vi "Import Export - Import from XML File.vi"(8 "error in":errorcluster, 10 "Configuration File Path":path, 11 "Item Ref in":T1 format="%.0x") -> (0 "error out":errorcluster, 3 "Item Ref out":T1 format="%.0x", 4 "xml string":string)   [LabVIEW 2017, in "PXImc System Explorer.lvlib"]
uses:
  PXImc System Explorer.lvlib
  <vilib>/NI Veristand/Custom Device API/Custom Device Item Ref.ctl
  <vilib>/NI/NI VeriStand Custom Device Import and Export Tool/ImportExport.lvlib
  <vilib>/NI VeriStand/Custom Device API/Custom Device API.lvlib
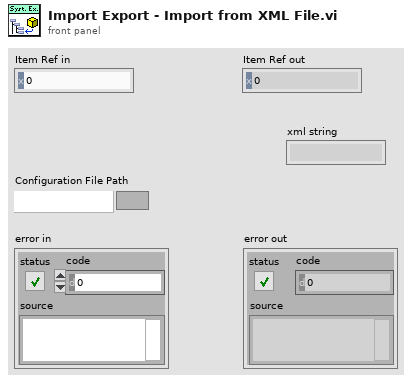
[diagram p1: front panel]
types:
  T1 = typedef "Custom Device API.lvlib/Custom Device Item Ref.ctl" = u64
  T2 = typedef "Advanced System Definition.lvlib/SysDef.Export.ctl" = cluster{"Version":string, "Tree":T3[]}
  T3 = typedef "Advanced System Definition.lvlib/TreeItem.ctl" = cluster{"Item Info":T4, "Parent Path":string[], "Properties":T9[]}
  T4 = typedef "Advanced System Definition.lvlib/TreeItem.Info.ctl" = cluster{"Name":string, "Description":string, "GUID":string, "Is Channel":bool, "Channel":T5, "Is Waveform":bool, "Waveform":T7}
  T5 = typedef "Custom Device API.lvlib/Custom Device Channel.ctl" = cluster{"Type":T6, "Units":string, "Default Value":dbl, "Faultable":bool, "Scalable":bool}
  T6 = typedef "Custom Device API.lvlib/Custom Device Channel Type.ctl" = enum16{"Input", "Output"}
  T7 = typedef "Custom Device API.lvlib/Custom Device Waveform.ctl" = cluster{"Data Type":T8, "Units":string}
  T8 = typedef "Custom Device API.lvlib/Custom Device Waveform DataType.ctl" = enum16{"Double", "Complex Double"}
  T9 = typedef "Advanced System Definition.lvlib/TreeItem.Property.ctl" = cluster{"Name":string, "Type":i32, "Value":variant}
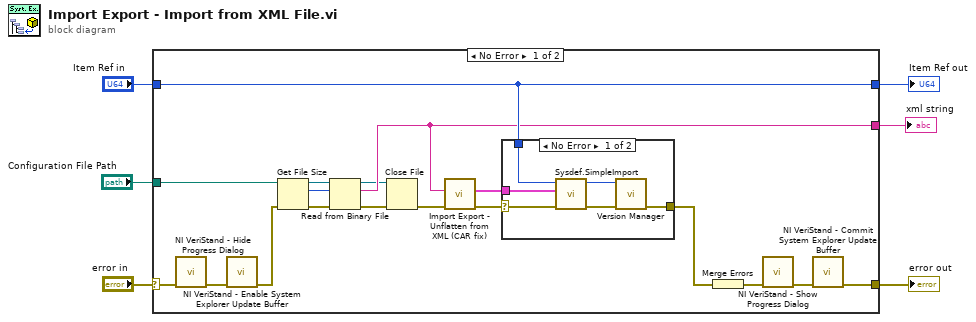
[diagram p0: block diagram]
diagram:
  n1 = case shown="No Error" "error in" {
    selector: "error in" -> [w11 w32]
    tunnel: [w9 w32] -> w5
    tunnel: [w24 w33] -> w4
    tunnel: "Item Ref in" -> [w24 w33]
    tunnel: "Configuration File Path" -> [w23 _]
    tunnel: [w22 _] -> w1
    frame No Error {
      n2 = call <vilib>:"NI VeriStand - Hide Progress Dialog.vi"("error in (no error)"=w11) -> ("error out"=w13:errorcluster)  [unwired: 10 in]
      n3 = call <vilib>:"NI VeriStand - Enable System Explorer Update Buffer.vi"("error in (no error)"=w13) -> ("error out"=w12:errorcluster)  [unwired: 10 in]
      n4 = Get File Size(file=w23, error in=w12) -> (refnum out=w18:refnum<file>, size (in bytes)=w19:i64, 0:w16:errorcluster)
      n5 = Read from Binary File(8:w16, 10:w19, 11:w18) -> (0:w15:errorcluster, 2:w22:string, 3:w17:refnum<file>)  [unwired: 3 in, 1 out]
      n6 = Close File(refnum=w17, error in=w15) -> (error out=w14:errorcluster)  [unwired: 1 out]
      n7 = call "Import Export - Unflatten from XML (CAR fix).vi"("Error In"=w14, "XML String In"=w22) -> ("Error Out"=w21:errorcluster, "Import"=w20:T2)  [unwired: 8 in]
      n8 = case shown="No Error" w21 {
        selector: w21 -> [w29 w31]
        tunnel: w20 -> [w30 _]
        tunnel: [w25 w31] -> w7
        tunnel: w24 -> [w28 _]
        frame No Error {
          n9 = call <vilib>:"Sysdef.SimpleImport.vi"("error in (no error)"=w29, "SysDef"=w30, "NodeID"=w28) -> ("error out"=w26:errorcluster, "NodeID out"=w27:u64)  [unwired: 7 in]
          n10 = call "Version Manager.vi"("error in (no error)"=w26, "Device Item Ref In in"=w27) -> ("error out"=w25:errorcluster)  [unwired: 8 in, 1 out]
        }
        frame Error {
        }
      }
      n11 = Merge Errors(w7) -> (w8:errorcluster)
      n12 = call <vilib>:"NI VeriStand - Show Progress Dialog.vi"("error in (no error)"=w8) -> ("error out"=w10:errorcluster)  [unwired: 10 in]
      n13 = call <vilib>:"NI VeriStand - Commit System Explorer Update Buffer.vi"("error in (no error)"=w10) -> ("error out"=w9:errorcluster)  [unwired: 10 in]
    }
    frame Error {
    }
  }
  "error out" <- w5
  "Item Ref out" <- w4
  "xml string" <- w1
